vi "Write.vi"(6 "Append Index":i32, 8 "error in (no error)":errorcluster, 9 "Notes":string, 10 "Data (Dictionary)":T1[](array[typedef]), 11 "Data.DAT in":refnum<class "LV-Data.DAT.lvclass">) -> (0 "error out":errorcluster, 3 "Data.DAT out":refnum<class "LV-Data.DAT.lvclass">, 5 "Path out":path)   [LabVIEW 2019, in "LV-Data.DAT.lvclass"]
uses:
  LV-Data.DAT.lvclass
  LV-Data/LV-Data.lvclass
  C:/Users/patrick/Documents/GitHub/LV-Data/src/LV-Data/LV-Data.lvclass
  Write DAT (2D).vi
  LV-Data/Typedefs/Dictionary--cluster.ctl
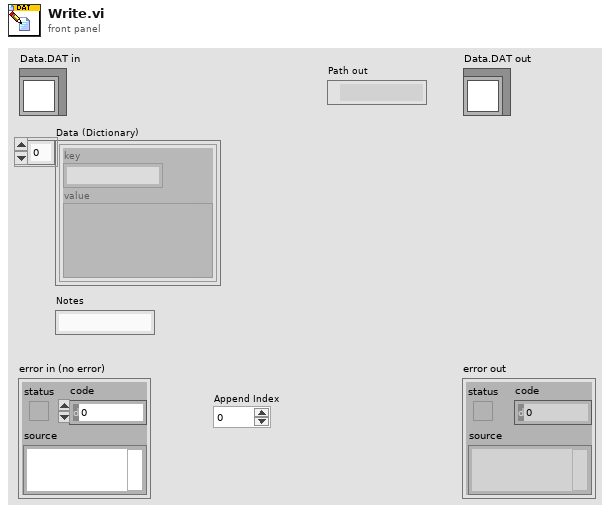
[diagram p1: front panel]
types:
  T1 = typedef "LV-Data.lvclass/Dictionary--cluster.ctl" = cluster{"key":string, "value":variant}
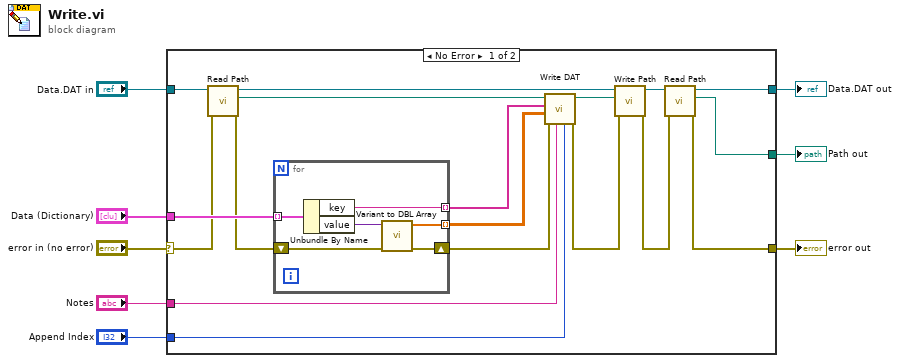
[diagram p0: block diagram]
diagram:
  n1 = case shown="No Error" "error in (no error)" {
    selector: "error in (no error)" -> [w17 w34]
    tunnel: [w12 w34] -> w7
    tunnel: "Data.DAT in" -> [w19 w33]
    tunnel: [w15 w33] -> w5
    tunnel: "Data (Dictionary)" -> [w23 _]
    tunnel: "Notes" -> [w20 _]
    tunnel: [w11 _] -> w2
    tunnel: "Append Index" -> [w18 _]
    frame No Error {
      n2 = call "Read Path.vi"("error in (no error)"=w17, "Data Save"=w19) -> ("error out"=w21:errorcluster, "Path"=w22:path, "Data Save out"=w24:refnum<class "LV-Data.DAT.lvclass">)  [unwired: 7 in]
      n3 = for {
        tunnel: w23 -> [w32] mode=indexing
        tunnel: [w31] -> w25 mode=indexing
        tunnel: [w29] -> w10 mode=indexing
        shift-right: [w27] -> w9
        shift-left: w21 -> [w28]
        n4 = Unbundle By Name(w32) -> ("key"=w31:string, "value"=w30:variant)
        n5 = call "Variant to DBL Array.vi"("error in (no error)"=w28, "Data (Variant)"=w30) -> ("error out"=w27:errorcluster, "1D Array"=w29:dbl[])  [unwired: 7 in, 1 out]
      }
      n6 = call-poly "Write DAT.vi"("Append (0=F)"=w18, "Comments"=w20, "error in"=w9, "Data"=w10, "Headers"=w25, "path"=w22) -> ("error out"=w26:errorcluster, "new file path"=w14:path)  [unwired: 4 in]
      n7 = call "Write Path.vi"("error in (no error)"=w26, "Path"=w14, "Data Save"=w24) -> ("error out"=w13:errorcluster, "Data Save out"=w16:refnum<class "LV-Data.DAT.lvclass">)  [unwired: 7 in]
      n8 = call "Read Path.vi"("error in (no error)"=w13, "Data Save"=w16) -> ("error out"=w12:errorcluster, "Path"=w11:path, "Data Save out"=w15:refnum<class "LV-Data.DAT.lvclass">)  [unwired: 7 in]
    }
    frame Error {
    }
  }
  "error out" <- w7
  "Data.DAT out" <- w5
  "Path out" <- w2
